vi "Base sp cluster selection for database_N.vi"(8 "error in":errorcluster, 10 "path":string="000.csv", 11 "Base":string) -> (0 "error out":errorcluster, 1 "Item":T1, 2 "element":string="000.csv", 3 "Base Species IDX":i32)   [LabVIEW 2018]
panel:
  out "R STD Level":dbl
  out "R Base Level":dbl
  out "Base Color":u32
  out "ex":string
  out "index":i32
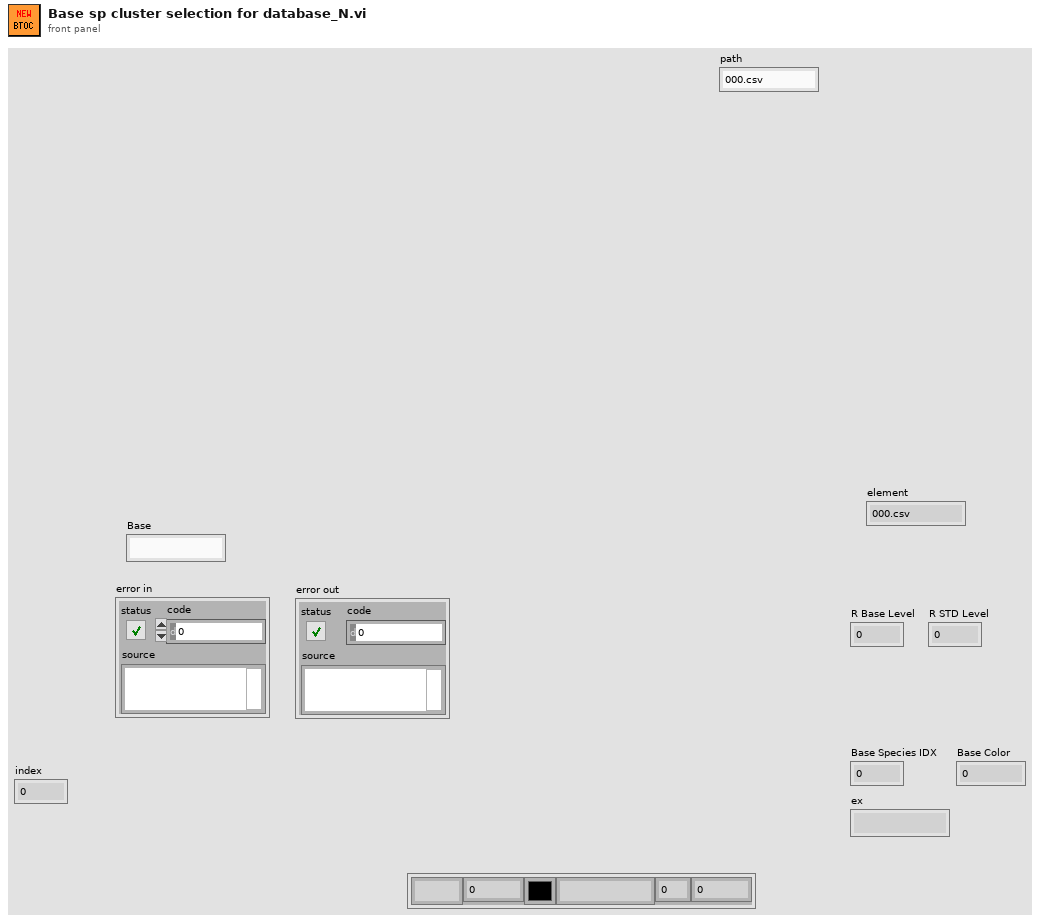
[diagram p1: front panel]
types:
  T1 = cluster{"Name":string, "Value":dbl, "Color":u32, "Name 2":string, "Value 2":dbl, "Value 3":dbl}
  T2 = cluster{"String":string, dbl, i32, "String":string, i32, dbl}
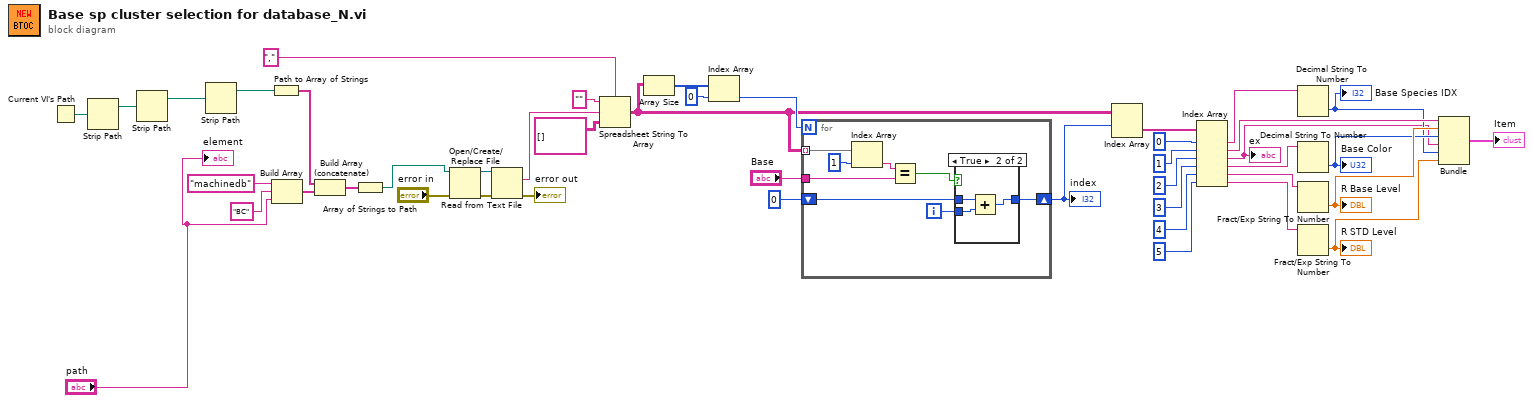
[diagram p0: block diagram]
diagram:
  n1 = Current VI's Path() -> (path=w44:path)
  n2 = Strip Path(path=w44) -> (stripped path=w43:path)  [unwired: 1 out]
  n3 = Strip Path(path=w43) -> (stripped path=w42:path)  [unwired: 1 out]
  n4 = Strip Path(path=w42) -> (stripped path=w41:path)  [unwired: 1 out]
  n5 = Path to Array of Strings(0:w41) -> (2:w38:string[])  [unwired: 1 out]
  n6 = Build Array("machinedb", "BC", "path") -> (w37:string[])
  n7 = Build Array (concatenate)(w38, w37) -> (w36:string[])
  n8 = Array of Strings to Path(0:w36) -> (2:w35:path)  [unwired: 1 in]
  n9 = Open/Create/Replace File(file path (use dialog)=w35, error in="error in") -> (refnum out=w32:refnum<file>, error out=w33:errorcluster)  [unwired: 4 in, 1 out]
  n10 = Read from Text File(file (use dialog)=w32, error in=w33) -> (text=w31:string, error out=→"error out":errorcluster)  [unwired: 2 in, 2 out]
  n11 = Spreadsheet String To Array(delimiter (Tab)=",", format string="", spreadsheet string=w31, array type (2D Dbl)=string[][] []) -> (array=w20:string[][])
  n12 = Array Size(array=w20) -> (size(s)=w26:i32[])
  n13 = Index Array(array=w26, index=0) -> (element=w24:i32)
  n14 = for {
    N: w24 -> [_]
    tunnel: w20 -> [w52] mode=indexing
    tunnel: "Base" -> [w49]
    shift-right: [w46] -> w21
    shift-left: 0 ("index") -> [w47]
    i -> [w45]
    n15 = Index Array(array=w52, index=1) -> (element=w50:string)
    n16 = Equal?(x=w50, y=w49) -> (x = y?=w48:bool)
    n17 = case shown="True" w48 {
      tunnel: [w53 w55] -> w46
      tunnel: w47 -> [w53 w54]
      tunnel: w45 -> [_ w56]
      frame False {
      }
      frame True {
        n18 = Add(x=w54, y=w56) -> (x+y=w55:i32)
      }
    }
  }
  "index" <- w21
  n19 = Index Array(array=w20, index (row)=w21) -> (element=w19:string[])  [unwired: 1 in]
  n20 = Index Array(array=w19, index #1=0 ("index"), index #2=1 ("index"), index #3=2 ("index"), index #4=3 ("index"), index #5=4 ("index"), index #6=5 ("index")) -> (element #1=w17:string, element #2=w15:string, element #3=w2:string, element #4=w9:string, element #5=w11:string, element #6=w6:string)
  "ex" <- w2
  n21 = Decimal String To Number(string=w17) -> (number=w5:i32)  [unwired: 2 in, 1 out]
  "Base Species IDX" <- w5
  n22 = Decimal String To Number(string=w9) -> (number=w8:i32)  [unwired: 2 in, 1 out]
  "Base Color" <- w8
  n23 = Fract/Exp String To Number(string=w11) -> (number=w10:dbl)  [unwired: 3 in, 1 out]
  "R Base Level" <- w10
  n24 = Fract/Exp String To Number(string=w6) -> (number=w3:dbl)  [unwired: 3 in, 1 out]
  "R STD Level" <- w3
  n25 = Bundle("String"=w15, w10, w8, "String"=w2, w5, w3) -> (→"Item":T2)  [unwired: 1 in]
  "element" <- "path"
